vi "Process.vi"(8 "error in":errorcluster, 11 "Instrument":refnum<class "Instrument.lvclass">) -> (0 "error out":errorcluster, 3 "Instrument out":refnum<class "Instrument.lvclass">)   [LabVIEW 2019, in "Instrument.lvlib" / "Instrument.lvclass"]
doc: "---------------------------------------------------------------\nJKI State Machine Objects™\nhttp://jki.net/state-machine-objects/\nCopyright (C) 2005-2015, JKI <info@jki.net>\nALL RIGHTS RESERVED"
uses:
  Instrument.lvclass
  C:/Program Files/National Instruments/LabVIEW 2019/vi.lib/JKI/JKI SMO/SMO/SMO.lvclass
  <userlib>/LevyLab/RemoteControl/RemoteControl/Typedefs/Message--Cluster.ctl
  <vilib>/JKI/JKI SMO/SMO/SMO.lvclass/SMO.ctl
  <vilib>/JKI/JKI SMO/SMO/Private/ReftoDVR--SMO.vi
  <vilib>/dlg_ctls.llb/Space Constant.vi
  <vilib>/AdvancedString/1D String Array to Delimited String.vi
  <userlib>/LevyLab/RemoteControl/RemoteControl/RemoteControl.lvclass
  <userlib>/LevyLab/Logger.Error/Logger.Error/Logger.Error.lvclass
  <userlib>/LevyLab/Logger.PGSQL/Logger.PGSQL/Logger.PGSQL.lvclass
  <vilib>/JKI/JKI SMO/SMO/SMO.lvclass
  <userlib>/LevyLab/Debug/Debug.lvlib
panel:
  out "State History":string
  out "Name":string
  out "Command":string
  # "1. Receives & processes commands from RemoteControl process\n2. Logs instrument settings to PGSQL using Logger process"
  # "INSTRUMENT"
  # "INSTRUMENT"
  # "For instructions on how to use the JKI State Machine Objects, examples and video tutorials, visit:\nhttp://jki.net/state-machine-objects/\n\nJKI State Machine Objects™\nhttp://jki.net/state-machine-objects/\nCopyright (C) 2005-2015, JKI <info@jki.net>\nALL RIGHTS RESERVED"
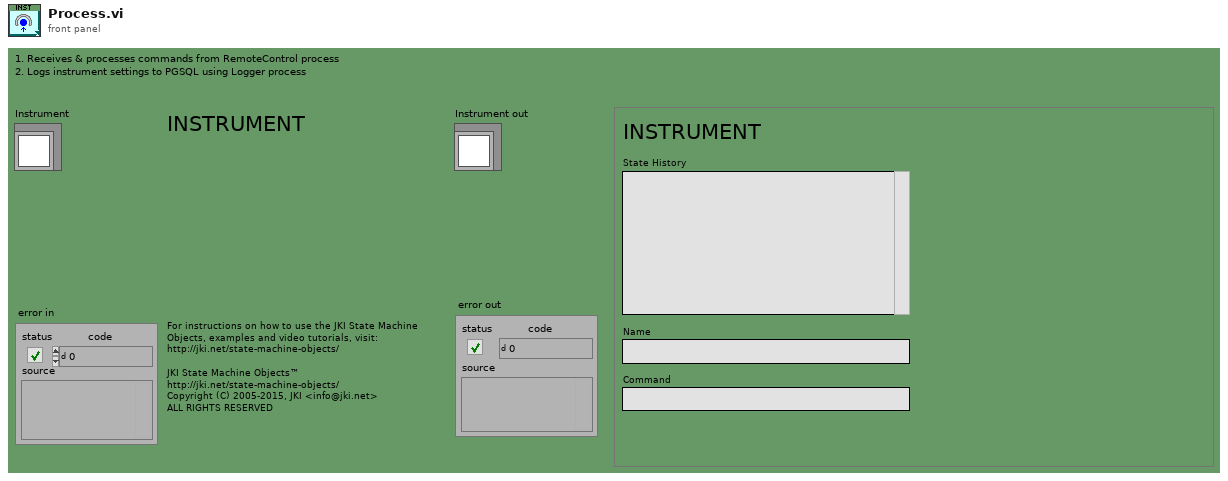
[diagram p1: front panel]
types:
  T1 = enum32{"invalid app kind", "Development System", "Run Time System", "Student Edition", "Embedded LabVIEW", "Evaluation", "Custom"}
  T2 = enum32{"Invalid", "Standard", "Closed", "Hidden", "Minimized", "Maximized"}
  T3 = typedef "RemoteControl.lvlib/RemoteControl.lvclass/Message--Cluster.ctl" = cluster{"Command":string, "Data":variant, "ID":string}
  T4 = typedef "Instrument.lvlib/Instrument.lvclass/Dependencies--Cluster.ctl" = cluster{"API":refnum<class "API.lvclass">, "Configuration":refnum<class "Configuration.lvclass">, "HAL":refnum<class "HAL.lvclass">, "DB-Logger":refnum<class "Logger.PGSQL.lvclass">, "Error-Logger":refnum<class "Logger.Error.lvclass">, "Remote-Control":refnum<class "RemoteControl.lvclass">}
  T5 = cluster{"Core":cluster{"Current VI Reference":refnum<vi>, "Close Panel on Exit?":bool, "Last Error":cluster{"error":errorcluster, "previous state":string, "remaining states":string}, "Shutdown?":bool}, "SMO":refnum<class "Instrument.lvclass">, "Dependencies":T4, "Message":T3}
  T6 = typedef "RemoteControl.lvclass/Message--Cluster.ctl" = cluster{"Command":string, "Data":variant, "ID":string}
  T7 = typedef "SMO.lvclass/SMOState --Enum.ctl" = enum16{"unknown", "Created", "Started", "Stopped"}
  T8 = cluster{"Current VI Reference":refnum<vi>, "Close Panel on Exit?":bool, "Last Error":cluster{"error":errorcluster, "previous state":string, "remaining states":string}, "Shutdown?":bool}
  T9 = typedef "Debug.lvlib/Attribute.Debug.lvclass/DebugBehavior.ctl" = enum16{"Normal", "Debug"}
  T10 = typedef "SMO.lvclass/Protected Events.ctl" = cluster{"StopProcesses":refnum<user-event>, "AbortProcesses":refnum<user-event>, "Config Changed":refnum<user-event>, "Dependency":refnum<user-event>}
  T11 = typedef "Instrument.lvlib/Instrument.lvclass/PrivateEvents--Cluster.ctl" = cluster{"MessageToProcess":refnum<user-event>, "LogData":refnum<user-event>, "LogDataMultiline":refnum<user-event>}
  T12 = typedef "RemoteControl.lvlib/RemoteControl.lvclass/PublicEvents--Cluster.ctl" = cluster{"SendMessageFromProcess":refnum<user-event>}
  T13 = typedef "SMO.lvclass/Public Events.ctl" = cluster{"Error":refnum<user-event>, "State":refnum<user-event>, "Reserve State":refnum<user-event>}
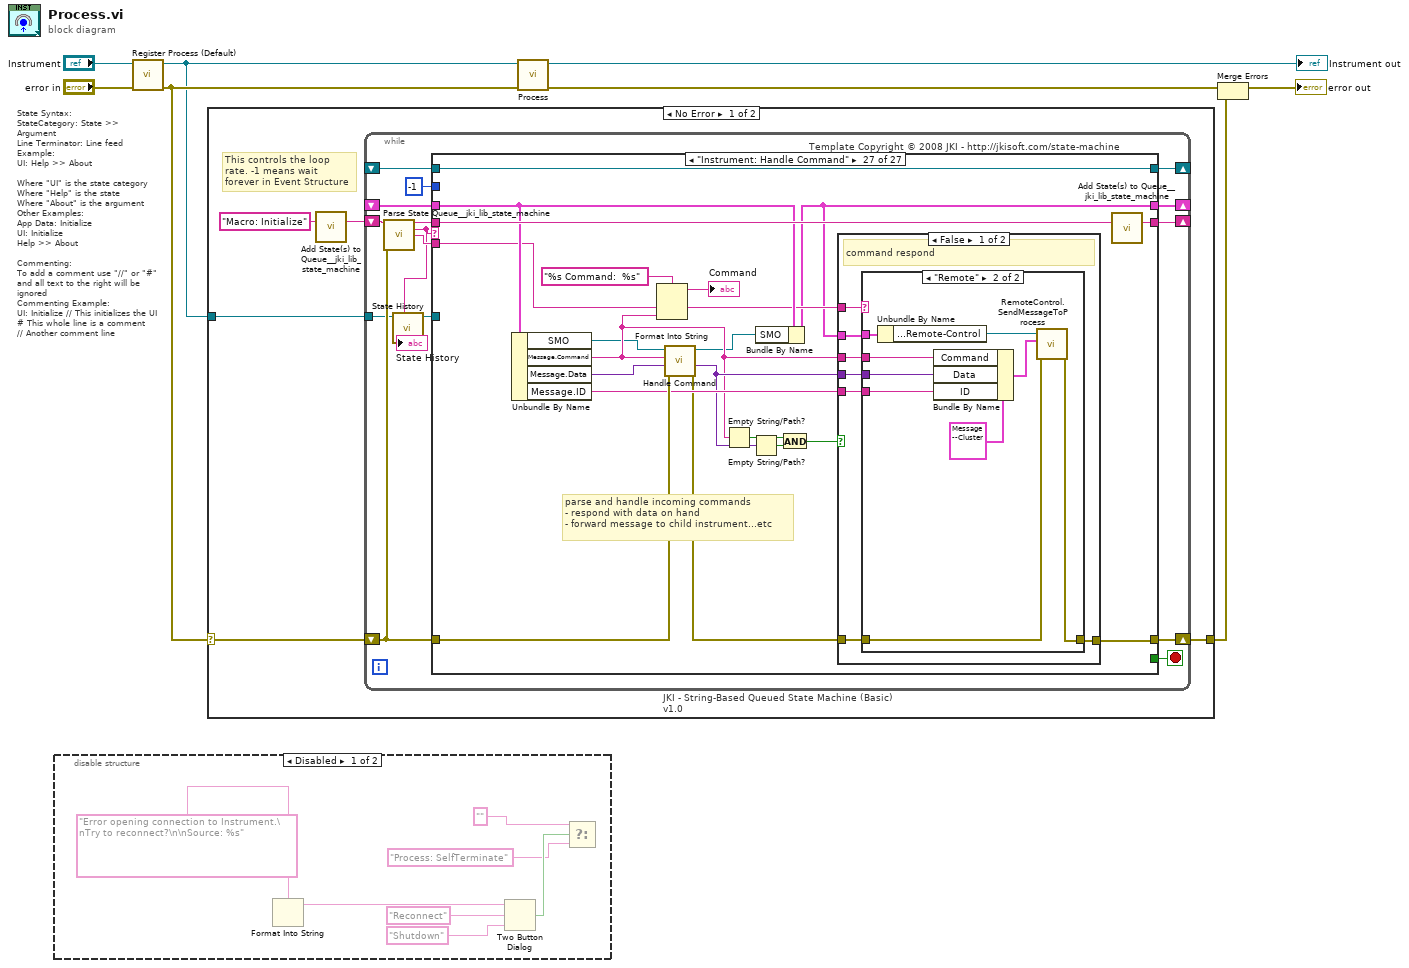
[diagram p0: block diagram]
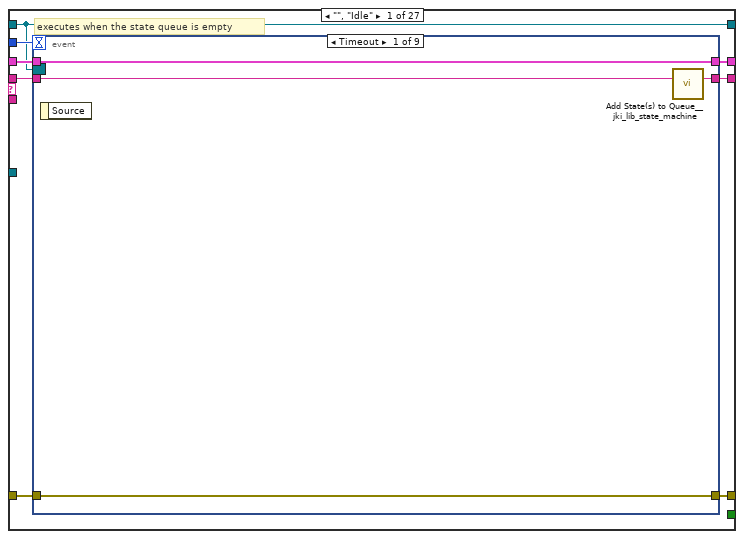
[diagram p3: hidden frame]
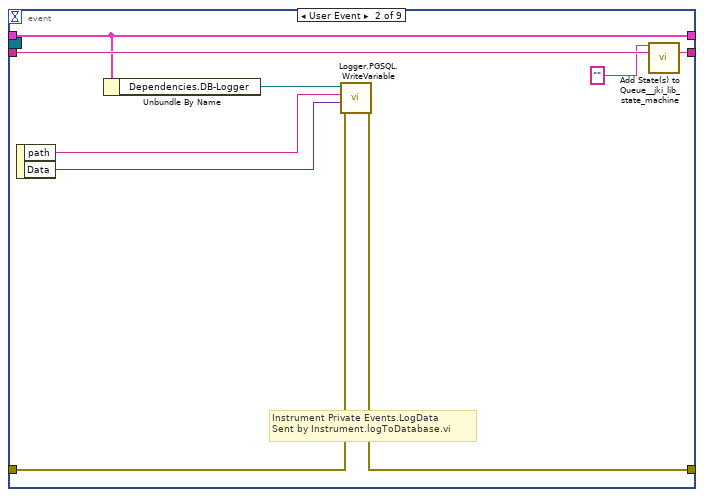
[diagram p4: hidden frame]
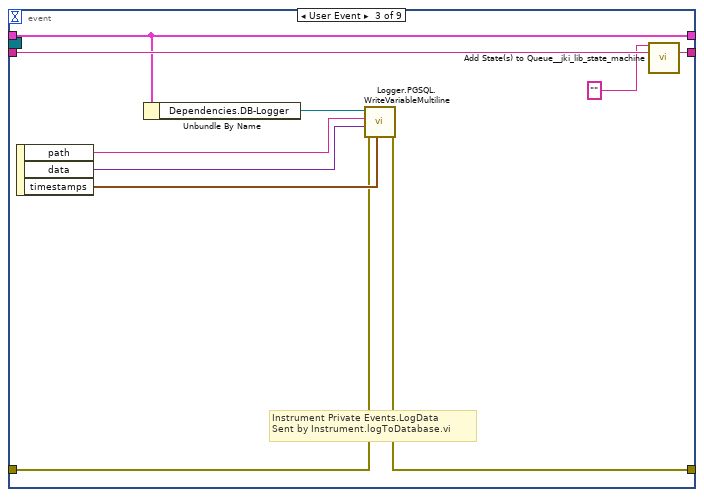
[diagram p5: hidden frame]
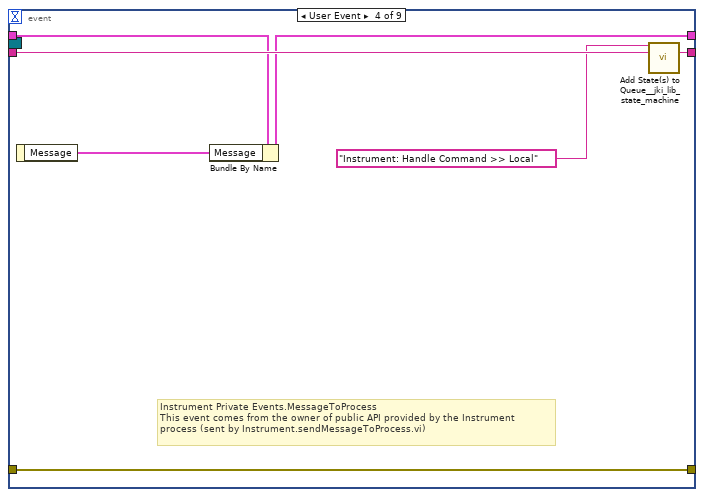
[diagram p6: hidden frame]
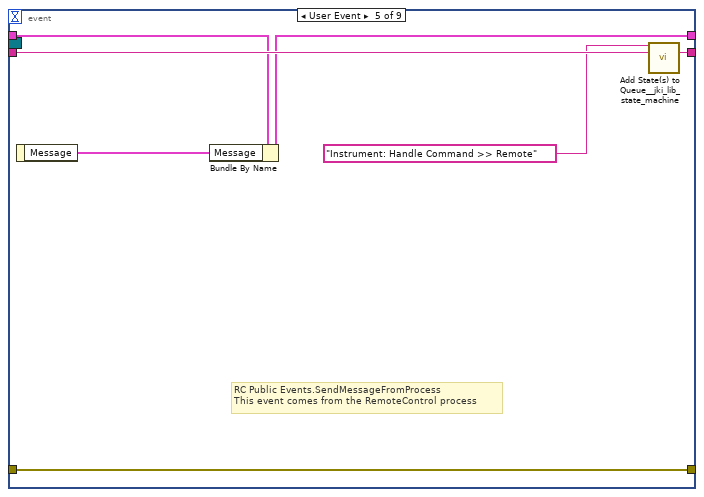
[diagram p7: hidden frame]
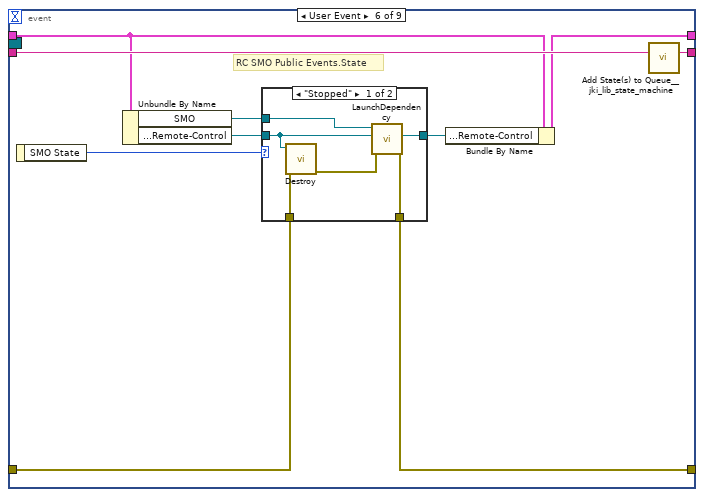
[diagram p8: hidden frame]
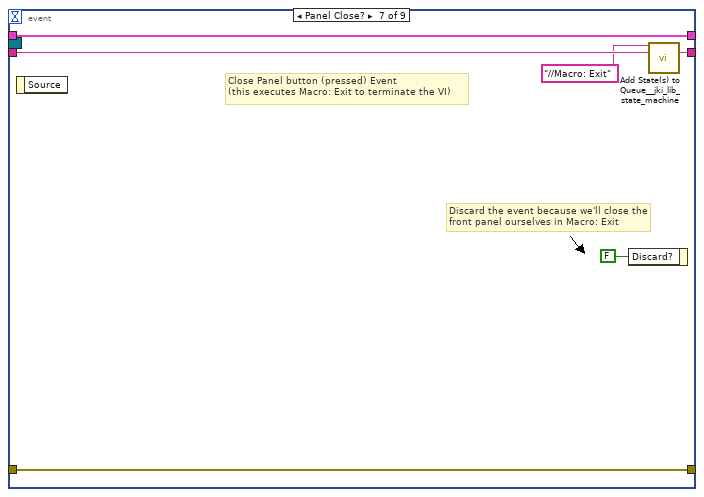
[diagram p10: hidden frame]
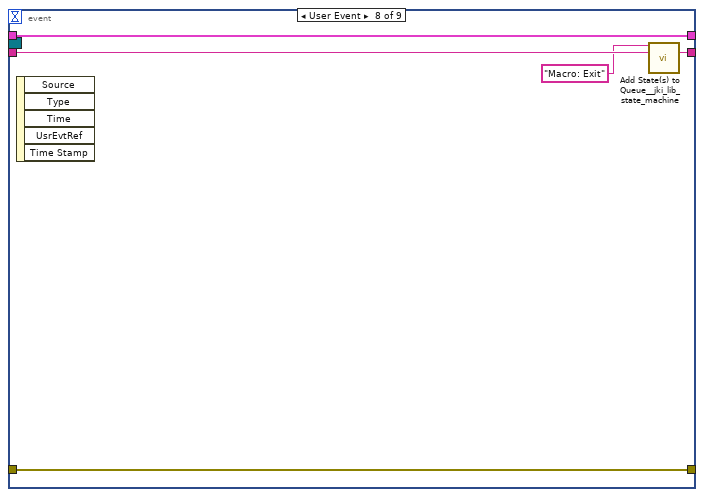
[diagram p11: hidden frame]
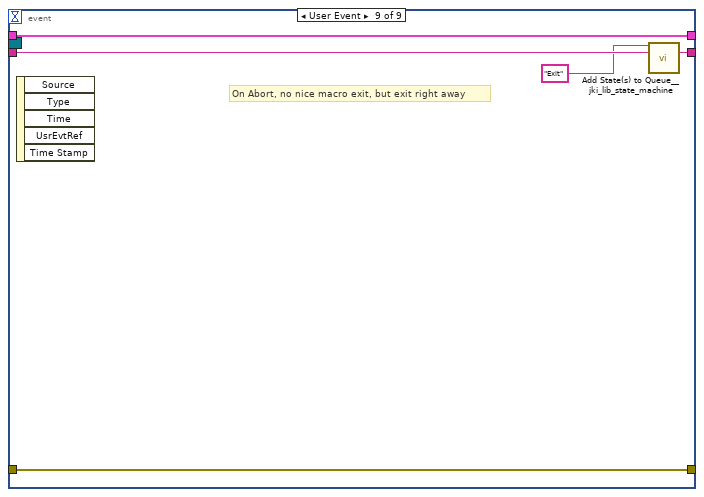
[diagram p12: hidden frame]
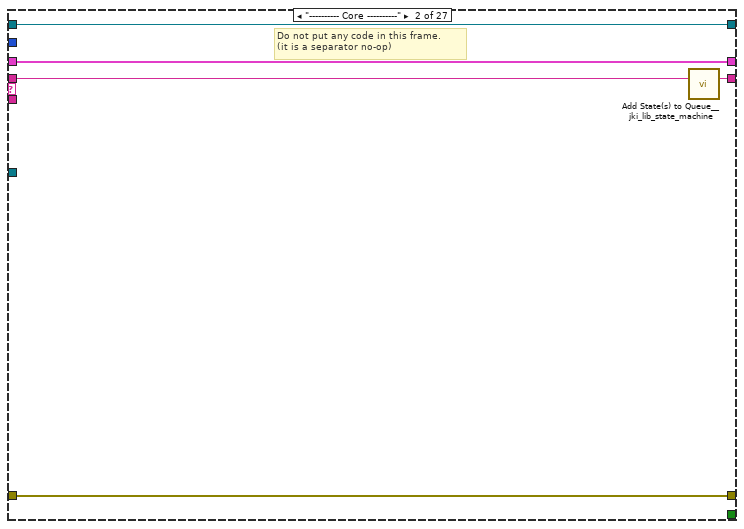
[diagram p13: hidden frame]
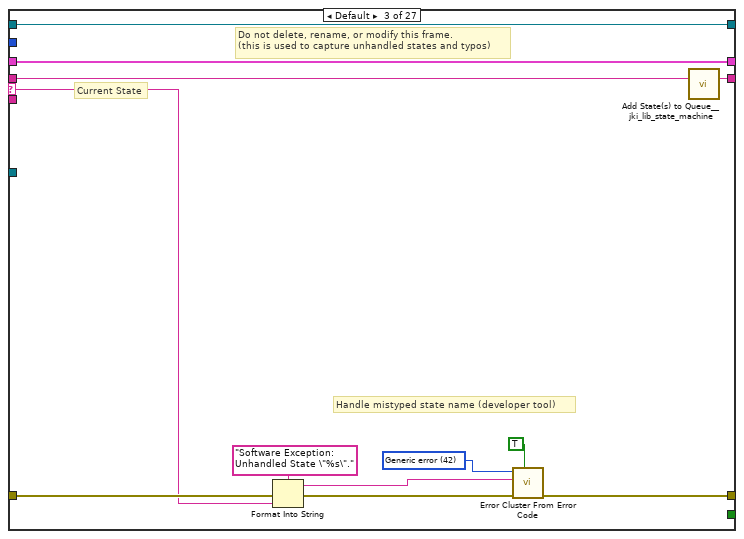
[diagram p14: hidden frame]
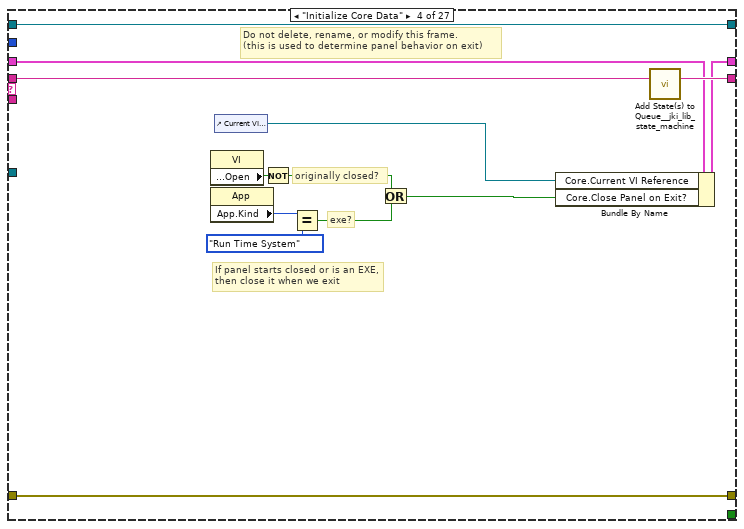
[diagram p15: hidden frame]
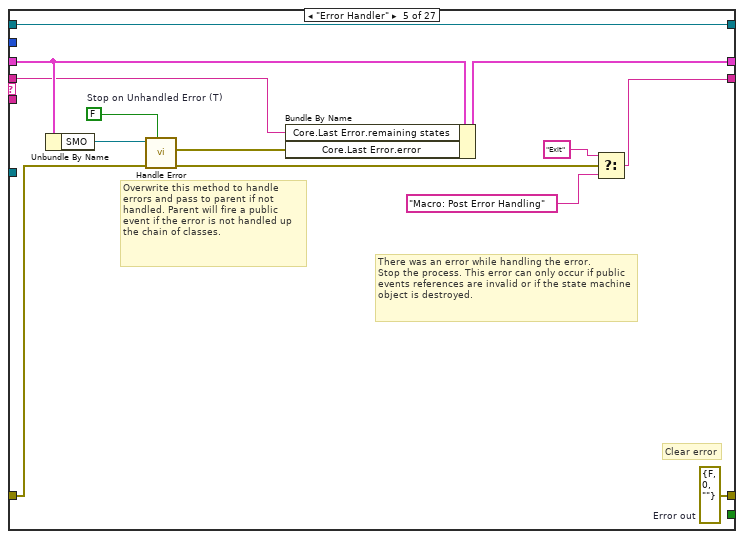
[diagram p16: hidden frame]
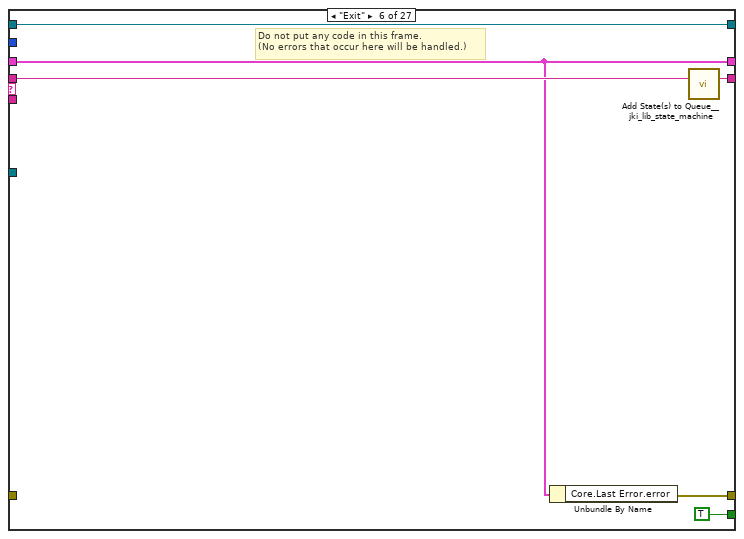
[diagram p17: hidden frame]
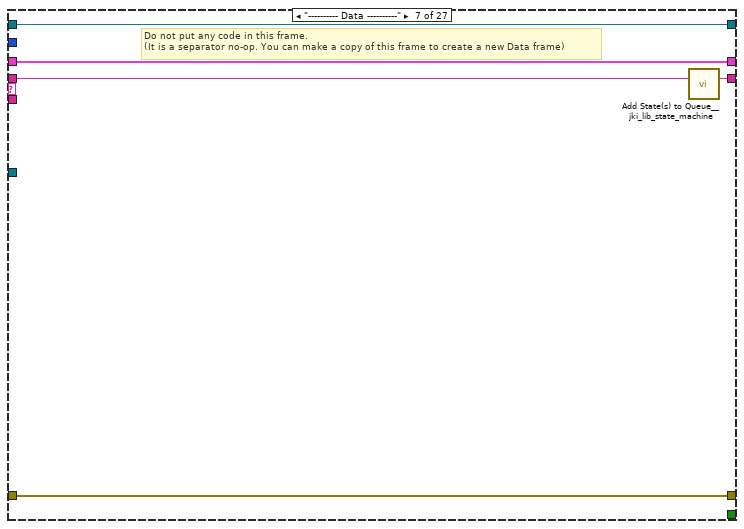
[diagram p18: hidden frame]
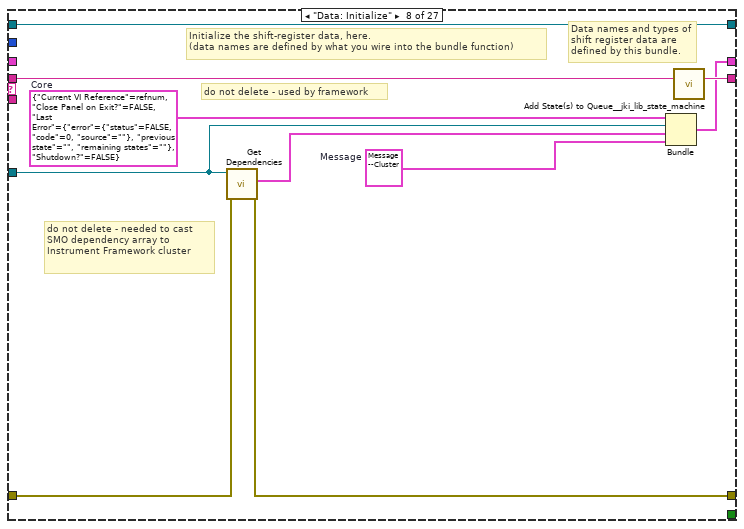
[diagram p19: hidden frame]
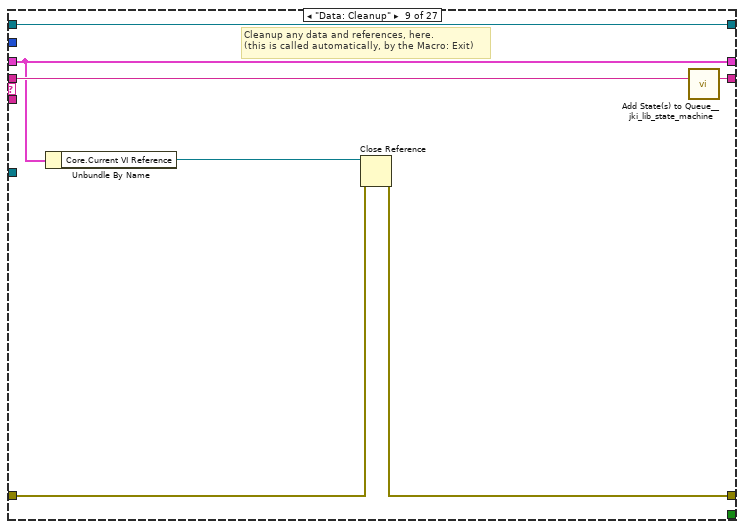
[diagram p20: hidden frame]
diagram:
  # "State Syntax:\nStateCategory: State >> Argument\nLine Terminator: Line feed\nExample:\nUI: Help >> About\n\nWhere \"UI\" is the state category\nWhere \"Help\" is the state\nWhere \"About\" is the argument\nOther Examples:\nApp Data: Initialize\nUI: Initialize\nHelp >> About\n\nCommenting:\nTo add a comment use \"//\" or \"#\" and all text to the right will be ignored\nCommenting Example:\nUI: Initialize // This initializes the UI\n# This whole line is a comment\n// Another comment line"
  n1 = disable-structure shown="Disabled" {
    frame Disabled {
      n2 = Format Into String(format string="Error opening connection to Instrument.\nTry to reconnect?\n\nSource: %s" ("message")) -> (resulting string=w9:string)  [unwired: 3 in, 1 out]
      n3 = Two Button Dialog(message=w9, 1:"Shutdown" ("F button name (\"Cancel\")"), 2:"Reconnect" ("T button name (\"OK\")")) -> (T button?=w13:bool)
      n4 = Select(t="" ("States to Execute"), s=w13, f="Process: SelfTerminate" ("States to Execute")) -> ()  [unwired: 1 out]
    }
    frame Enabled {
    }
  }
  n5 = call <vilib>:"Register Process (Default).vi"("error in (no error)"="error in", "SMO"="Instrument") -> ("error out"=w5:errorcluster, "SelfRef"=w4:refnum<class "Instrument.lvclass">)  [unwired: 8 in]
  n6 = case shown="No Error" w5 {
    selector: w5 -> [w17 w443]
    tunnel: w4 -> [w18 _]
    tunnel: [w16 w443] -> w1
    frame No Error {
      # "This controls the loop rate. -1 means wait forever in Event Structure"
      n7 = call <vilib>:"Add State(s) to Queue__jki_lib_state_machine.vi"("State(s) in (\"\")"="Macro: Initialize") -> ("States Out"=w20:string)  [unwired: 14 in]
      n8 = while "JKI - String-Based Queued State Machine (Basic) v1.0" {
        shift-right: [w30] -> _
        shift-left: _ -> [w29]
        shift-right: [w33] -> w16
        shift-left: w17 -> [w27]
        shift-right: [w32] -> _
        shift-left: w20 -> [w34]
        tunnel: w18 -> [w21]
        shift-right: [w26] -> _
        shift-left: _ -> [w25]
        stop <- w31 stop-if-true
        # "Template Copyright © 2008 JKI - http://jkisoft.com/state-machine"
        n9 = call <vilib>:"Parse State Queue__jki_lib_state_machine.vi"("State Queue"=w34, "Error In (no error)"=w27) -> ("Remaining States"=w36:string, "Current State"=w24:string, "Arguments"=w35:string)  [unwired: 11 in]
        n10 = call <userlib>:"State History.vi"("Current State"=w24, "SMO"=w21) -> ("SMO"=w22:refnum<class "Instrument.lvclass">, "History"=→"State History":string)  [unwired: 8 in]
        n11 = case shown="\"Instrument: Handle Command\"" w24 {
          selector: w24 -> [_ _ w122 _ _ _ _ _ _ _ _ _ _ _ _ _ _ _ _ _ _ _ _ _ _ _ _]
          tunnel: w36 -> [w44 w120 w126 w145 w147 w164 w169 w179 w186 w191 w201 w208 w224 w260 w265 w274 w290 w294 w321 w331 w342 w351 w356 w387 w393 w398 w418]
          tunnel: w35 -> [_ _ _ _ _ _ _ _ _ _ _ w202 w218 w254 _ _ _ _ _ _ _ _ _ _ _ _ w401]
          tunnel: w29 -> [w42 w117 w124 w136 w156 w160 w166 _ w181 w188 w198 w206 w220 w257 w262 w268 w276 w297 w310 w328 w339 w346 w353 w385 w391 w396 w403]
          tunnel: [w41 w118 w128 w142 w157 w159 w167 w171 w182 w189 w192 w203 w221 w253 w263 w267 w288 w301 w309 w329 w333 w343 w354 w383 w389 w394 w408] -> w33
          tunnel: w27 -> [w40 w118 w127 w142 w148 _ w167 w172 w183 w189 w195 w204 w222 w253 w263 w267 w288 w301 w308 w329 w334 w344 w354 w381 w389 w394 w415]
          tunnel: [w43 w119 w125 w144 w152 w163 w168 w178 w185 w190 w200 w207 w223 w259 w264 w273 w289 w295 w320 w330 w341 w350 w355 w386 w392 w397 w417] -> w32
          tunnel: [_ _ _ _ _ TRUE _ _ _ _ _ _ _ _ _ _ _ _ _ _ _ _ _ _ _ _ _] -> w31
          tunnel: [w39 w117 w124 w143 w155 w160 w166 w170 w181 w188 w198 w206 w220 w257 w262 w268 w277 w298 w311 w328 w339 w345 w353 w385 w391 w396 w399] -> w30
          tunnel: -1 ("Timeout") -> [w38 _ _ _ _ _ _ _ _ _ _ _ _ _ _ _ _ _ _ _ _ _ _ _ _ _ _]
          tunnel: [w37 w116 w121 w133 w158 w161 w165 w177 w180 w187 w199 w205 w217 w258 w261 w272 w283 w302 w319 w327 w340 w349 w352 w384 w390 w395 w416] -> w26
          tunnel: w25 -> [w37 w116 w121 w133 w158 w161 w165 w177 w180 w187 w199 w205 w217 w258 w261 w272 w283 w302 w319 w327 w340 w349 w352 _ w390 w395 w416]
          tunnel: w22 -> [_ _ _ _ _ _ _ w173 _ _ _ _ _ _ _ _ _ _ _ _ _ _ _ _ _ _ _]
          frame "", "Idle" {
            # "executes when the state queue is empty"
            n12 = event shown="[0] Timeout" {
              selector: w37 -> [_ _ _ _ _ _ _ _ _]
              dyn-events: _ -> [_ _ _ _ _ _ _ _ _]
              timeout: w38 -> [_ _ _ _ _ _ _ _ _]
              tunnel: w44 -> [w48 w57 w67 w74 w81 w91 w105 w110 w115]
              tunnel: [w47 w56 w66 w73 w80 w90 w104 w109 w114] -> w43
              tunnel: w42 -> [w45 w49 w58 w71 w78 w87 w102 w107 w112]
              tunnel: [w46 w51 w60 w72 w79 w84 w103 w108 w113] -> w41
              tunnel: w40 -> [w46 w50 w59 w72 w79 w85 w103 w108 w113]
              tunnel: [w45 w49 w58 w70 w77 w86 w102 w107 w112] -> w39
              event Timeout {
                n13 = event-data() -> ()  [unwired: 1 in, 1 out]
                n14 = call <vilib>:"Add State(s) to Queue__jki_lib_state_machine.vi"("State(s) in (\"\")"=w48) -> ("States Out"=w47:string)  [unwired: 14 in]
              }
              event User Event {
                # "Instrument Private Events.LogData\nSent by Instrument.logToDatabase.vi"
                n15 = event-data() -> ("path"=w52:string, "Data"=w53:variant)  [unwired: 1 in]
                n16 = Unbundle By Name(w49) -> ("Dependencies.DB-Logger"=w54:refnum<class "Logger.PGSQL.lvclass">)
                n17 = call <userlib>:"Logger.PGSQL.WriteVariable.vi"("error in (no error)"=w50, "Data"=w53, "Address"=w52, "Logger"=w54) -> ("error out"=w51:errorcluster)  [unwired: 6 in, 1 out]
                n18 = call <vilib>:"Add State(s) to Queue__jki_lib_state_machine.vi"("State(s) in Front (\"\")"="" ("State(s) in Front (\"\")"), "State(s) in (\"\")"=w57) -> ("States Out"=w56:string)  [unwired: 13 in]
              }
              event User Event {
                # "Instrument Private Events.LogData\nSent by Instrument.logToDatabase.vi"
                n19 = event-data() -> ("path"=w63:string, "data"=w62:variant, "timestamps"=w61:timestamp[])  [unwired: 1 in]
                n20 = Unbundle By Name(w58) -> ("Dependencies.DB-Logger"=w64:refnum<class "Logger.PGSQL.lvclass">)
                n21 = call <userlib>:"Logger.PGSQL.WriteVariableMultiline.vi"("Timestamps"=w61, "error in (no error)"=w59, "Data"=w62, "Address"=w63, "Logger"=w64) -> ("error out"=w60:errorcluster)  [unwired: 5 in, 1 out]
                n22 = call <vilib>:"Add State(s) to Queue__jki_lib_state_machine.vi"("State(s) in Front (\"\")"="" ("State(s) in Front (\"\")"), "State(s) in (\"\")"=w67) -> ("States Out"=w66:string)  [unwired: 13 in]
              }
              event User Event {
                # "Instrument Private Events.MessageToProcess\nThis event comes from the owner of public API provided by the Instrument\nprocess (sent by Instrument.sendMessageToProcess.vi)"
                n23 = event-data() -> ("Message"=w69:T3)  [unwired: 1 in]
                n24 = Bundle By Name(cluster=w71, "Message"=w69) -> (w70:T5)
                n25 = call <vilib>:"Add State(s) to Queue__jki_lib_state_machine.vi"("State(s) in Front (\"\")"="Instrument: Handle Command >> Local" ("State(s) in Front (\"\")"), "State(s) in (\"\")"=w74) -> ("States Out"=w73:string)  [unwired: 13 in]
              }
              event User Event {
                # "RC Public Events.SendMessageFromProcess\nThis event comes from the RemoteControl process"
                n26 = event-data() -> ("Message"=w76:T6)  [unwired: 1 in]
                n27 = Bundle By Name(cluster=w78, "Message"=w76) -> (w77:T5)
                n28 = call <vilib>:"Add State(s) to Queue__jki_lib_state_machine.vi"("State(s) in Front (\"\")"="Instrument: Handle Command >> Remote" ("State(s) in Front (\"\")"), "State(s) in (\"\")"=w81) -> ("States Out"=w80:string)  [unwired: 13 in]
              }
              event User Event {
                # "RC SMO Public Events.State"
                n29 = event-data() -> ("SMO State"=w82:T7)  [unwired: 1 in]
                n30 = Unbundle By Name(w87) -> ("SMO"=w83:refnum<class "Instrument.lvclass">, "Dependencies.Remote-Control"=w89:refnum<class "RemoteControl.lvclass">)
                n31 = case shown="\"Stopped\"" w82 {
                  tunnel: w89 -> [w92 w99]
                  tunnel: [w97 w99] -> w88
                  tunnel: w85 -> [w94 w98]
                  tunnel: [w96 w98] -> w84
                  tunnel: w83 -> [w95 _]
                  frame "Stopped" {
                    n32 = call <vilib>:"Destroy.vi"("error in (no error)"=w94, "SMO"=w92) -> ("error out"=w93:errorcluster)  [unwired: 9 in]
                    n33 = call <vilib>:"LaunchDependency.vi"("error in (no error)"=w93, "Dependency Type"=w92, "SMO in"=w95) -> ("error out"=w96:errorcluster, "Dependency Reference"=w97:refnum<class "RemoteControl.lvclass">)  [unwired: 5 in, 2 out]
                  }
                  frame Default {
                  }
                }
                n34 = Bundle By Name(cluster=w87, "Dependencies.Remote-Control"=w88) -> (w86:T5)
                n35 = call <vilib>:"Add State(s) to Queue__jki_lib_state_machine.vi"("State(s) in (\"\")"=w91) -> ("States Out"=w90:string)  [unwired: 14 in]
              }
              event Panel Close? {
                # "Discard the event because we'll close the front panel ourselves in Macro: Exit"
                # "Close Panel button (pressed) Event\n(this executes Macro: Exit to terminate the VI)"
                n36 = event-data() -> ()  [unwired: 1 in, 1 out]
                n37 = event-data("Discard?"=FALSE) -> ()  [unwired: 1 in, 1 out]
                n38 = call <vilib>:"Add State(s) to Queue__jki_lib_state_machine.vi"("State(s) in Front (\"\")"="//Macro: Exit", "State(s) in (\"\")"=w105) -> ("States Out"=w104:string)  [unwired: 13 in]
              }
              event User Event {
                n39 = event-data() -> ()  [unwired: 1 in, 5 out]
                n40 = call <vilib>:"Add State(s) to Queue__jki_lib_state_machine.vi"("State(s) in Front (\"\")"="Macro: Exit", "State(s) in (\"\")"=w110) -> ("States Out"=w109:string)  [unwired: 13 in]
              }
              event User Event {
                # "On Abort, no nice macro exit, but exit right away"
                n41 = event-data() -> ()  [unwired: 1 in, 5 out]
                n42 = call <vilib>:"Add State(s) to Queue__jki_lib_state_machine.vi"("State(s) in Front (\"\")"="Exit", "State(s) in (\"\")"=w115) -> ("States Out"=w114:string)  [unwired: 13 in]
              }
            }
          }
          frame "---------- Core ----------" {
            # "Do not put any code in this frame.\n(it is a separator no-op)"
            n43 = call <vilib>:"Add State(s) to Queue__jki_lib_state_machine.vi"("State(s) in (\"\")"=w120) -> ("States Out"=w119:string)  [unwired: 14 in]
          }
          frame Default {
            w131 = 42 items=["No error", "Argument error", "Memory is full", "Out of zone", "End of file", "File already open", "Generic file I/O error", "File not found", "File permission error", "Disk is full", "Duplicate path", "Too many files open", "System feature not enabled", "Resource file not found", "Cannot add resource", "Resource not found", "Image not found", "Image memory error", "Pen does not exist", "Config type invalid", "Config token not found", "Config parse error", "Config memory error", "Bad external code format", "Bad external code offset", "External code not present", "Null window", "Destroy window error", "Null menu", "Print aborted", "Bad print record", "Print driver error", "Windows error during printing", "Memory error during printing", "Print dialog error", "Generic print error", "Invalid device refnum", "Device not found", "Device parameter error", "Device unit error", "Cannot open device", "Device call aborted", "Generic error", "Cancelled by user", "Object ID too low", "Object ID too high", "Object not in heap", "Unknown heap", "Unknown object (invalid DefProc)", "Unknown object (DefProc not in table)", "Message out of range", "Invalid (null) method", "Unknown message", "Manager call not supported", "Bad address", "Network operation in progress", "Network operation timed out", "Connection is busy", "Network attribute not supported", "Network error", "Address in use", "System out of memory", "Connection aborted", "Connection refused", "Not connected", "Already connected", "Connection closed", "Initialization error (interapplication manager)", "Bad occurrence", "Wait on unbound occurrence handler", "Occurrence queue overflow", "Datalog type conflict", "Unused", "Unrecognized type (interapplication manager)", "Memory corrupt", "Failed to make temporary DLL", "Old CIN version", "Drag socket not found", "Failed to load drop-object", "Failed to register OLE object", "Failed to release OLE object", "Format specifier type mismatch", "Unknown format specifier", "Too few format specifiers", "Too many format specifiers", "Scan failed", "Newer CIN version", "Error converting to variant", "Runtime menu error", "Password tampered", "Variant attribute not found", "Incompatible variant data type", "Event data is not available", "Event Store is not present", "Occurrence is not found", "Event Queue is not created", "Event info is not available", "Refnum passed is NULL", "Error retrieving Class GUID", "Error retrieving CoClass GUID", "Error retrieving TypeLib GUID.", "Bad built application magic bytes.", "Specific driver is different from the specific driver associated with the Logical Name.", "There is no session opened to the class driver.", "Max Error", "MAX - Error with config objects", "MAX - Error loading configuration", "MAX - Group not supported"]
            # "Current State"
            # "Do not delete, rename, or modify this frame.\n(this is used to capture unhandled states and typos)"
            # "Handle mistyped state name (developer tool)"
            n44 = Format Into String(format string="Software Exception: Unhandled State \"%s\"." ("message"), error in=w127, w122) -> (resulting string=w130:string, error out=w129:errorcluster)  [unwired: 1 in]
            n45 = call <vilib>:"Error Cluster From Error Code.vi"("show call chain? (False)"=TRUE, "error in (no error)"=w129, "error message (\"\")"=w130, "error code (0)"=w131) -> ("error out"=w128:errorcluster)  [unwired: 5 in]
            n46 = call <vilib>:"Add State(s) to Queue__jki_lib_state_machine.vi"("State(s) in (\"\")"=w126) -> ("States Out"=w125:string)  [unwired: 14 in]
          }
          frame "Initialize Core Data" {
            # "Do not delete, rename, or modify this frame.\n(this is used to determine panel behavior on exit)"
            # "originally closed?"
            # "exe?"
            # "If panel starts closed or is an EXE, then close it when we exit"
            n47 = property class="VI"() -> ("Front Panel.Open"=w141:bool)  [unwired: 2 in, 2 out]
            n48 = property class="App"() -> ("App.Kind"=w140:T1)  [unwired: 2 in, 2 out]
            n49 = control-ref of="Current VI Reference"() -> (w134:refnum<vi>)
            n50 = Not(x=w141) -> (.not. x?=w138:bool)
            n51 = Equal?(x=w140, y=T1."Run Time System" ("Application:Kind")) -> (x = y?=w137:bool)
            n52 = Or(x=w138, y=w137) -> (x .or. y?=w135:bool)
            n53 = Bundle By Name(cluster=w136, "Core.Current VI Reference"=w134, "Core.Close Panel on Exit?"=w135) -> (w143:T5)
            n54 = call <vilib>:"Add State(s) to Queue__jki_lib_state_machine.vi"("State(s) in (\"\")"=w145) -> ("States Out"=w144:string)  [unwired: 14 in]
          }
          frame "Error Handler" {
            w153 = FALSE  # Stop on Unhandled Error (T)
            w157 = errorcluster {"status"=FALSE, "code"=0, "source"=""}  # Error out
            # "Clear error"
            # "There was an error while handling the error.\nStop the process. This error can only occur if public events references are invalid or if the state machine object is destroyed."
            # "Overwrite this method to handle errors and pass to parent if not handled. Parent will fire a public event if the error is not handled up the chain of classes."
            n55 = Unbundle By Name(w156) -> ("SMO"=w149:refnum<class "Instrument.lvclass">)
            n56 = call-dynamic "Handle Error.vi"("Stop on Unhandled Error (T)"=w153, "error in"=w148, "SMO"=w149) -> ("handling error"=w150:errorcluster, "Unhandled error"=w151:errorcluster)  [unwired: 6 in, 1 out]
            n57 = Bundle By Name(cluster=w156, "Core.Last Error.remaining states"=w147, "Core.Last Error.error"=w151) -> (w155:T5)
            n58 = Select(t="Exit", s=w150, f="Macro: Post Error Handling" ("State")) -> (s? t:f=w152:string)
          }
          frame "Exit" {
            # "Do not put any code in this frame.\n(No errors that occur here will be handled.)"
            n59 = Unbundle By Name(w160) -> ("Core.Last Error.error"=w159:errorcluster)
            n60 = call <vilib>:"Add State(s) to Queue__jki_lib_state_machine.vi"("State(s) in (\"\")"=w164) -> ("States Out"=w163:string)  [unwired: 14 in]
          }
          frame "---------- Data ----------" {
            # "Do not put any code in this frame.\n(It is a separator no-op. You can make a copy of this frame to create a new Data frame)"
            n61 = call <vilib>:"Add State(s) to Queue__jki_lib_state_machine.vi"("State(s) in (\"\")"=w169) -> ("States Out"=w168:string)  [unwired: 14 in]
          }
          frame "Data: Initialize" {
            w175 = T3 {"Command"="", "Data"=variant(string ""), "ID"=""}  # Message
            w176 = T8 {"Current VI Reference"=refnum, "Close Panel on Exit?"=FALSE, "Last Error"={"error"={"status"=FALSE, "code"=0, "source"=""}, "previous state"="", "remaining states"=""}, "Shutdown?"=FALSE}  # Core
            # "do not delete - needed to cast SMO dependency array to Instrument Framework cluster"
            # "do not delete - used by framework"
            # "Data names and types of shift register data are defined by this bundle."
            # "Initialize the shift-register data, here.\n(data names are defined by what you wire into the bundle function)"
            n62 = call "Get Dependencies.vi"("error in (no error)"=w172, "Instrument in"=w173) -> ("error out"=w171:errorcluster, "Dependencies"=w174:T4)  [unwired: 7 in, 1 out]
            n63 = Bundle("Core"=w176, "SMO"=w173, "Dependencies"=w174, "Message"=w175) -> (w170:T5)  [unwired: 1 in]
            n64 = call <vilib>:"Add State(s) to Queue__jki_lib_state_machine.vi"("State(s) in (\"\")"=w179) -> ("States Out"=w178:string)  [unwired: 14 in]
          }
          frame "Data: Cleanup" {
            # "Cleanup any data and references, here.\n(this is called automatically, by the Macro: Exit)"
            n65 = Unbundle By Name(w181) -> ("Core.Current VI Reference"=w184:refnum<vi>)
            n66 = Close Reference(reference=w184, error in (no error)=w183) -> (error out=w182:errorcluster)
            n67 = call <vilib>:"Add State(s) to Queue__jki_lib_state_machine.vi"("State(s) in (\"\")"=w186) -> ("States Out"=w185:string)  [unwired: 14 in]
          }
          frame "---------- UI ----------" {
            # "Do not put any code in this frame.\n(It is a separator no-op. You can make a copy of this frame to create a new UI frame)"
            n68 = call <vilib>:"Add State(s) to Queue__jki_lib_state_machine.vi"("State(s) in (\"\")"=w191) -> ("States Out"=w190:string)  [unwired: 14 in]
          }
          frame "UI: Initialize" {
            # "Initialize the User Interface, here.\n(this is called automatically, by the Macro: Init)"
            n69 = Unbundle By Name(w198) -> ("SMO"=w197:refnum<class "Instrument.lvclass">)
            n70 = call <vilib>:"GetName.vi"("error in (no error)"=w195, "SMO"=w197) -> ("error out"=w193:errorcluster, "Name"=→"Name":string)  [unwired: 6 in, 2 out]
            n71 = call <userlib>:"Fit VI window to Largest Dec__ogtk.vi"("error in (no error)"=w193, "border spacing (2 px)"=0) -> ("error out"=w192:errorcluster)  [unwired: 4 in, 1 out]
            n72 = call <vilib>:"Add State(s) to Queue__jki_lib_state_machine.vi"("State(s) in (\"\")"=w201) -> ("States Out"=w200:string)  [unwired: 14 in]
          }
          frame "UI: Cursor Set" {
            # "Argument"
            # "Initialize the User Interface, here.\n(this is called automatically, by the Macro: Init)"
            n73 = disable-structure shown="Default" {
              disable-tunnel: w204 -> [w209 w212]
              disable-tunnel: [w209 w211] -> w203
              disable-tunnel: w202 -> [_ w210]
              frame condition #0 {
              }
              frame condition #1 (active) {
                n74 = case shown="\"Busy\"" w210 {
                  tunnel: w212 -> [w214 w216]
                  tunnel: [w213 w215] -> w211
                  frame "Idle", Default {
                    n75 = call <vilib>:"Unset Busy.vi"("error in (no error)"=w214) -> ("error out"=w213:errorcluster)  [unwired: 10 in]
                  }
                  frame "Busy" {
                    n76 = call <vilib>:"Set Busy.vi"("error in (no error)"=w216) -> ("error out"=w215:errorcluster)  [unwired: 9 in, 1 out]
                  }
                }
              }
            }
            n77 = call <vilib>:"Add State(s) to Queue__jki_lib_state_machine.vi"("State(s) in (\"\")"=w208) -> ("States Out"=w207:string)  [unwired: 14 in]
          }
          frame "UI: Front Panel State" {
            # "Argument"
            # "Set Front Panel Open or Closed\n(Usage: \"UI: Front Panel State >> Open|Close\")"
            n78 = Unbundle By Name(w220) -> ("Core.Current VI Reference"=w219:refnum<vi>)
            n79 = disable-structure shown="Default" {
              disable-tunnel: w222 -> [w228 w251]
              disable-tunnel: [w227 w251] -> w221
              disable-tunnel: w219 -> [w226 _]
              disable-tunnel: w218 -> [w225 _]
              frame condition #0 (active) {
                n80 = case shown="\"Close\"" w225 {
                  tunnel: w228 -> [w232 w245]
                  tunnel: [w234 w246] -> w227
                  tunnel: w226 -> [w233 w243]
                  frame "Open", Default {
                    n81 = property class="VI"(reference=w233, error in=w232) -> (reference out=w230:refnum<vi>, error out=w231:errorcluster, "FP.State"=w229:T2)
                    n82 = case shown="Default" w229 {
                      tunnel: [w237 w240] -> w234
                      tunnel: w231 -> [w236 w240]
                      tunnel: w230 -> [w235 _]
                      frame "Closed" {
                        n83 = invoke class="VI" method="FP.Open"(reference=w235, error in=w236, "Activate"=TRUE, "State"=T2."Standard") -> (error out=w237:errorcluster)  [unwired: 1 in, 4 out]
                      }
                      frame Default {
                      }
                    }
                  }
                  frame "Close" {
                    n84 = property class="VI"(reference=w243, error in=w245) -> (reference out=w242:refnum<vi>, error out=w244:errorcluster, "FP.State"=w241:T2)
                    n85 = case shown="Default" w241 {
                      tunnel: [w247 w250] -> w246
                      tunnel: w244 -> [w247 w249]
                      tunnel: w242 -> [_ w248]
                      frame "Invalid", "Closed" {
                      }
                      frame Default {
                        n86 = invoke class="VI" method="FP.Close"(reference=w248, error in=w249) -> (error out=w250:errorcluster)  [unwired: 1 in, 2 out]
                      }
                    }
                  }
                }
              }
              frame condition #1 {
              }
            }
            n87 = call <vilib>:"Add State(s) to Queue__jki_lib_state_machine.vi"("State(s) in (\"\")"=w224) -> ("States Out"=w223:string)  [unwired: 14 in]
          }
          frame "UI: Wait" {
            n88 = Scan From String(format string="%d", input string=w254, default 1=u32 0 ("default value 1")) -> (output 1=w252:u32)  [unwired: 2 in, 3 out]
            n89 = Wait (ms)(milliseconds to wait=w252) -> ()  [unwired: 1 out]
            n90 = call <vilib>:"Add State(s) to Queue__jki_lib_state_machine.vi"("State(s) in (\"\")"=w260) -> ("States Out"=w259:string)  [unwired: 14 in]
          }
          frame "---------- Macro ----------" {
            # "Do not put any code in this frame.\n(It is a separator no-op. You can make a copy of this frame to create a new Macro frame)"
            n91 = call <vilib>:"Add State(s) to Queue__jki_lib_state_machine.vi"("State(s) in (\"\")"=w265) -> ("States Out"=w264:string)  [unwired: 14 in]
          }
          frame "Macro: Initialize" {
            # "Initialization Macro\n(This is called once, when the VI starts)"
            n92 = call <vilib>:"Add State(s) to Queue__jki_lib_state_machine.vi"("State(s) in Front (\"\")"="Data: Initialize\nInitialize Core Data\nEvents: Register", "State(s) in (\"\")"="Process: Sync", "State(s) at Back (\"\")"="UI: Initialize\nUI: Front Panel State >> Close\nMacro: Debug") -> ("States Out"=w270:string)  [unwired: 12 in]
            n93 = call <vilib>:"Add State(s) to Queue__jki_lib_state_machine.vi"("State(s) in Front (\"\")"=w270, "State(s) in (\"\")"=w274) -> ("States Out"=w273:string)  [unwired: 13 in]
          }
          frame "Macro: Exit" {
            # "Exit Macro\n(This is called once, when the VI exits)"
            n94 = Unbundle By Name(w276) -> ("Core.Close Panel on Exit?"=w287:bool)
            n95 = Select(t="UI: Front Panel State >> Close", s=w287, f="") -> (s? t:f=w285:string)
            n96 = Bundle By Name(cluster=w276, "Core.Shutdown?"=TRUE) -> (w277:T5)
            n97 = call <vilib>:"Add State(s) to Queue__jki_lib_state_machine.vi"("State(s) in Front (\"\")"="Data: Cleanup\nEvents: Unregister", "State(s) in (\"\")"="Process: Sync", "State(s) at Back (\"\")"="Exit") -> ("States Out"=w280:string)  [unwired: 12 in]
            n98 = call <vilib>:"Add State(s) to Queue__jki_lib_state_machine.vi"("State(s) in (\"\")"=w285, "State(s) at Back (\"\")"=w280) -> ("States Out"=w284:string)  [unwired: 13 in]
            n99 = call <vilib>:"Add State(s) to Queue__jki_lib_state_machine.vi"("State(s) in Front (\"\")"=w284, "State(s) in (\"\")"=w290) -> ("States Out"=w289:string)  [unwired: 13 in]
          }
          frame "Macro: Post Error Handling" {
            # "Clear Last Error?"
            n100 = Unbundle By Name(w297) -> ("Core.Last Error.remaining states"=w299:string, "Core.Shutdown?"=w300:bool)
            n101 = Unbundle By Name(w297) -> ("Core.Last Error.error"=w292:errorcluster)
            n102 = case shown="False" FALSE {
              tunnel: w292 -> [w303 _]
              tunnel: [w303 _] -> w291
              frame False {
              }
              frame True {
              }
            }
            n103 = case shown="True" w300 {
              tunnel: w299 -> [w304 w306]
              tunnel: [w304 w305] -> w296
              frame False {
                # "These are the remaining states (at the moment the error occured). States can be altered according to business logic."
                # "NOT SHUTTING DOWN"
              }
              frame True {
                # "Developer can decide to alter the states but should be aware that during the shutdown process, there are certain states that must be run for the SMO to properly shut itself (and this process) down. As such, one can add states to perform additional clean-ups, but should append the remaining state to be executed."
                # "SHUTTING DOWN"
                n104 = call <vilib>:"Add State(s) to Queue__jki_lib_state_machine.vi"("State(s) in (\"\")"=w306) -> ("States Out"=w305:string)  [unwired: 14 in]
              }
            }
            n105 = Bundle By Name(cluster=w297, "Core.Last Error.error"=w291) -> (w298:T5)
            n106 = call <vilib>:"Add State(s) to Queue__jki_lib_state_machine.vi"("State(s) in Front (\"\")"=w296, "State(s) in (\"\")"=w294) -> ("States Out"=w295:string)  [unwired: 13 in]
          }
          frame "Macro: Debug" {
            # "exe?"
            # "If pane is an EXE, then close it when we exit"
            # "Macro: Debug\n(get debug behavior, determine UI and determine shutdown behavior)"
            n107 = Unbundle By Name(w310) -> ("Core.Close Panel on Exit?"=w313:bool, "SMO"=w318:refnum<class "Instrument.lvclass">)
            n108 = property class="App"() -> ("App.Kind"=w316:T1)  [unwired: 2 in, 2 out]
            n109 = Equal?(x=w316, y=T1."Run Time System" ("Application:Kind")) -> (x = y?=w312:bool)
            n110 = call <userlib>:"Get Debug Mode.vi"("error in (no error)"=w308, "SMO"=w318) -> ("error out"=w309:errorcluster, "Behavior"=w317:T9)  [unwired: 7 in, 1 out]
            n111 = case shown="\"Normal\", Default" w317 {
              tunnel: [w322 w324] -> w314
              tunnel: w313 -> [w322 _]
              tunnel: w312 -> [_ w326]
              tunnel: [_ "UI: Front Panel State >> Open\nUI: Wait >> 1000"] -> w307
              frame "Normal", Default {
                # "respect core.close"
              }
              frame "Debug" {
                # "keep panel open\nunless exe"
                n112 = Or(x=w326, y=FALSE) -> (x .or. y?=w324:bool)
              }
            }
            n113 = Bundle By Name(cluster=w310, "Core.Close Panel on Exit?"=w314) -> (w311:T5)
            n114 = call <vilib>:"Add State(s) to Queue__jki_lib_state_machine.vi"("State(s) in Front (\"\")"=w307, "State(s) in (\"\")"=w321) -> ("States Out"=w320:string)  [unwired: 13 in]
          }
          frame "---------- Process ----------" {
            # "Template Separator\n(You can make a copy of, or modify, this frame)"
            n115 = call <vilib>:"Add State(s) to Queue__jki_lib_state_machine.vi"("State(s) in (\"\")"=w331) -> ("States Out"=w330:string)  [unwired: 14 in]
          }
          frame "Process: Sync" {
            n116 = Unbundle By Name(w339) -> ("SMO"=w335:refnum<class "Instrument.lvclass">)
            n117 = call <vilib>:"WaitOnProcessSync.vi"("error in (no error)"=w334, "SMO"=w335) -> ("error out"=w333:errorcluster, "Don't run?"=w338:bool)  [unwired: 7 in, 1 out]
            n118 = Select(t="Data: Cleanup\nEvents: Unregister\nExit", s=w338, f="") -> (s? t:f=w332:string)
            n119 = call <vilib>:"Add State(s) to Queue__jki_lib_state_machine.vi"("State(s) in Front (\"\")"=w332, "State(s) in (\"\")"=w342) -> ("States Out"=w341:string)  [unwired: 13 in]
          }
          frame "Process: SelfTerminate" {
            # "Template Separator\n(You can make a copy of, or modify, this frame)"
            n120 = Unbundle By Name(w346) -> ("SMO"=w348:refnum<class "Instrument.lvclass">)
            n121 = call <vilib>:"SelfTerminate.vi"("error in (no error)"=w344, "SMO in"=w348) -> ("error out"=w343:errorcluster, "SMO out"=w347:refnum<class "Instrument.lvclass">)  [unwired: 8 in]
            n122 = Bundle By Name(cluster=w346, "SMO"=w347) -> (w345:T5)
            n123 = call <vilib>:"Add State(s) to Queue__jki_lib_state_machine.vi"("State(s) in (\"\")"=w351) -> ("States Out"=w350:string)  [unwired: 14 in]
          }
          frame "---------- Events ----------" {
            # "Template Separator\n(You can make a copy of, or modify, this frame)"
            n124 = call <vilib>:"Add State(s) to Queue__jki_lib_state_machine.vi"("State(s) in (\"\")"=w356) -> ("States Out"=w355:string)  [unwired: 14 in]
          }
          frame "Events: Register" {
            n125 = Unbundle By Name(w385) -> ("SMO"=w380:refnum<class "Instrument.lvclass">, "Dependencies.Remote-Control"=w379:refnum<class "RemoteControl.lvclass">, "Dependencies.DB-Logger"=w374:refnum<class "Logger.PGSQL.lvclass">, "Dependencies.Error-Logger"=w375:refnum<class "Logger.Error.lvclass">)
            n126 = call <vilib>:"GetProtectedEvents.vi"("SMO"=w380) -> ("error out"=w382:errorcluster, "SMO Protected Events"=w370:T10, "SMO out"=w373:refnum<class "Instrument.lvclass">)  [unwired: 8 in]
            n127 = call "Instrument.GetPrivateEvents.vi"("Instrument"=w373) -> ("error out"=w369:errorcluster, "Instrument Private Events"=w367:T11)  [unwired: 8 in, 1 out]
            n128 = call <userlib>:"RemoteControl.GetPublicEvents.vi"("RemoteControl"=w379) -> ("error out"=w368:errorcluster, "RC Public Events"=w366:T12, "RemoteControl out"=w372:refnum<class "RemoteControl.lvclass">)  [unwired: 8 in]
            n129 = call <vilib>:"GetPublicEvents.vi"("SMO"=w372) -> ("error out"=w378:errorcluster, "Public Events"=w365:T13)  [unwired: 8 in, 1 out]
            n130 = call <vilib>:"GetPublicEvents.vi"("SMO"=w374) -> ("error out"=w377:errorcluster, "Public Events"=w363:T13)  [unwired: 8 in, 1 out]
            n131 = call <vilib>:"GetPublicEvents.vi"("SMO"=w375) -> ("error out"=w376:errorcluster, "Public Events"=w360:T13)  [unwired: 8 in, 1 out]
            n132 = call "Rename RC SMO Private Events.vi"("error in (no error)"=w378, "Public Events"=w365) -> ("error out"=w357:errorcluster, "RC SMO Public Events"=w364:T13)  [unwired: 8 in]
            n133 = call "Rename PGSQL SMO Private Events.vi"("error in (no error)"=w377, "Public Events"=w363) -> ("error out"=w358:errorcluster, "PGSQL SMO Public Events"=w362:T13)  [unwired: 8 in]
            n134 = call "Rename Error SMO Private Events.vi"("error in (no error)"=w376, "Public Events"=w360) -> ("error out"=w361:errorcluster, "RC SMO Public Events"=w359:T13)  [unwired: 8 in]
            n135 = register-events(w370, w367, w366, w364, w362, w359) -> (reference out=w384:refnum<event-registration>, error out=w371:errorcluster)  [unwired: 2 in]
            n136 = Merge Errors(w371, w357, w358, w361, w368, w369, w382, w381) -> (w383:errorcluster)
            n137 = call <vilib>:"Add State(s) to Queue__jki_lib_state_machine.vi"("State(s) in (\"\")"=w387) -> ("States Out"=w386:string)  [unwired: 14 in]
          }
          frame "Events: Unregister" {
            n138 = Unregister For Events(event registration refnum=w390, error in=w389) -> (error out=w388:errorcluster)
            n139 = call <vilib>:"Clear Errors.vi"("error in (no error)"=w388) -> ()  [unwired: 5 in, 2 out]
            n140 = call <vilib>:"Add State(s) to Queue__jki_lib_state_machine.vi"("State(s) in (\"\")"=w393) -> ("States Out"=w392:string)  [unwired: 14 in]
          }
          frame "---------- Instrument ----------" {
            n141 = call <vilib>:"Add State(s) to Queue__jki_lib_state_machine.vi"("State(s) in (\"\")"=w398) -> ("States Out"=w397:string)  [unwired: 14 in]
          }
          frame "Instrument: Handle Command" {
            # "parse and handle incoming commands\n- respond with data on hand\n- forward message to child instrument...etc"
            n142 = Unbundle By Name(w403) -> ("SMO"=w400:refnum<class "Instrument.lvclass">, "Message.Command"=w404:string, "Message.Data"=w413:variant, "Message.ID"=w414:string)
            n143 = Format Into String(format string="%s Command:  %s", w401, w404) -> (resulting string=→"Command":string)  [unwired: 2 in, 1 out]
            n144 = call-dynamic "Handle Command.vi"("error in (no error)"=w415, "params in"=w413, "command"=w404, "Instrument in"=w400) -> ("error out"=w407:errorcluster, "processed data"=w409:variant, "Instrument out"=w402:refnum<class "Instrument.lvclass">)  [unwired: 4 in, 1 out]
            n145 = Empty String/Path?(string/path=w404) -> (empty?=w412:bool)
            n146 = Empty String/Path?(string/path=w409) -> (empty?=w411:bool)
            n147 = Bundle By Name(cluster=w403, "SMO"=w402) -> (w399:T5)
            n148 = And(x=w412, y=w411) -> (x .and. y?=w410:bool)
            n149 = case shown="False" w410 {
              tunnel: w407 -> [w422 w442]
              tunnel: w409 -> [w424 _]
              tunnel: w414 -> [w425 _]
              tunnel: [w421 w442] -> w408
              tunnel: w404 -> [w423 _]
              tunnel: w401 -> [w420 _]
              tunnel: w399 -> [w419 _]
              frame False {
                # "command respond"
                n150 = case shown="\"Remote\"" w420 {
                  tunnel: w425 -> [w430 w436]
                  tunnel: w424 -> [w426 w435]
                  tunnel: w423 -> [w432 w437]
                  tunnel: w422 -> [w431 w441]
                  tunnel: [w429 w440] -> w421
                  tunnel: w419 -> [w428 w434]
                  frame "Local", Default {
                    n151 = Unbundle By Name(w428) -> ("SMO"=w427:refnum<class "Instrument.lvclass">)
                    n152 = call "Instrument.sendMessageFromProcess.vi"("ID"=w430, "error in (no error)"=w431, "Data"=w426, "Command"=w432, "Instrument"=w427) -> ("error out"=w429:errorcluster)  [unwired: 5 in, 1 out]
                  }
                  frame "Remote" {
                    n153 = Unbundle By Name(w434) -> ("Dependencies.Remote-Control"=w433:refnum<class "RemoteControl.lvclass">)
                    n154 = Bundle By Name(cluster=T3 {"Command"="", "Data"=variant(string ""), "ID"=""} ("Message"), "Command"=w437, "Data"=w435, "ID"=w436) -> (w438:T3)
                    n155 = call <userlib>:"RemoteControl.SendMessageToProcess.vi"("error in (no error)"=w441, "Message"=w438, "RemoteControl"=w433) -> ("error out"=w440:errorcluster)  [unwired: 7 in, 1 out]
                  }
                }
              }
              frame True {
              }
            }
            n156 = call <vilib>:"Add State(s) to Queue__jki_lib_state_machine.vi"("State(s) in (\"\")"=w418) -> ("States Out"=w417:string)  [unwired: 14 in]
          }
        }
      }
    }
    frame Error {
    }
  }
  n157 = call-parent "Process.vi"("error in"=w5, "SMO"=w4) -> ("error out"=w2:errorcluster, "SMO out"=→"Instrument out":refnum<class "Instrument.lvclass">)  [unwired: 8 in]
  n158 = Merge Errors(w2, w1) -> (→"error out":errorcluster)
